vi "Cyclic Scheduler.vi"(8 "error in (no error)":errorcluster, 9 "timeout ms":i32=100, 11 "Variables":T1={"Process Ref"=refnum, "Comm Ref"=refnum, "Data Refs"={"ProtectionsAndCounters.Ref"=refnum, "Signals.Ref"=refnum, "Status.Ref"=refnum, "Overrides"=refnum, "IncomingSignals.Ref"=refnum, "CtrandProtctnVld.Ref"=refnum, "RcvTime.Ref"=refnum, "TimeDiff.Ref"=refnum, "IncomingProtCtr.Ref"=refnum}, "Settings"={"Name"="", "Priority"=0, "XNET Settings"={"Database"="", "Cluster"="", "Port"="", "Baud rate [Bd]"=0, "Termination"=0, "CAN I/O Mode"=0, "FD Baud rate [Bd]"=500000, "Priority"=100, "Use Legacy"=FALSE, "FD ISO Mode"=0, "Default Max Counter Value"=0.0, "Default Protect Type"=enum."Arb ID + Bytes Checksum with Inversion", "Include All Channels"=FALSE, "Scheduler Bucket Size"=10, "Scheduler Offset"=3}, "FPGA Session"=0, "Outgoing CAN Session"="", "Outgoing Cyclic Frame Count"=0, "Outgoing Cyclic Frames"=[], "Outgoing Event Frame Count"=0, "Outgoing Event Frames"=[], "Incoming CAN Session"="", "Incoming Frame Count"=0, "Incoming Frames"=[], "Incoming Values"={"Signal Values"=[], "Signal Invalid Values"=[], "ProtCtr Sig Values"=[], "Timestamps"=[], "Time Differences"=[], "IDs"=[]}}, "Stream Refs"={"Addon"="", "Port"="", "Filter Ref"=refnum, "Default Filter"={"ID Filters"=[], "Direction Filter"=enum."Tx/Rx", "Type Filter"=enum."All"}, "Port Settings"={"Mode"=0, "Baud Rate"=0, "Termination"=0, "FD ISO Mode"=0, "FD Baud Rate"=0}}, "Cyclic Scheduler Queue"=refnum, "Cyclic Scheduler FIFO"=refnum} {"Stream Refs"."Port Settings"."FD ISO Mode" items=["ISO", "Non ISO", "ISO Legacy"]; "Stream Refs"."Port Settings"."Termination" items=["Off", "On"]; "Stream Refs"."Port Settings"."Mode" items=["CAN 2.0", "CAN FD", "CAN FD+BRS"]; "Settings"."XNET Settings"."FD ISO Mode" items=["ISO", "Non ISO", "ISO Legacy"]; "Settings"."XNET Settings"."CAN I/O Mode" items=["CAN 2.0", "CAN FD", "CAN FD+BRS"]; "Settings"."XNET Settings"."Termination" items=["Off", "On"]}) -> (0 "error out":errorcluster)   [LabVIEW 2023, in "Protection and Counter Addon Engine.lvlib"]
uses:
  Protection and Counter Addon Engine.lvlib
  <vilib>/NI/NIVS Inline Async API/_VS Inline Async API/Process/Process.lvclass
  <vilib>/NI/NI VeriStand Addon Network Comm/Engine/VeriStand Comm.lvclass
  <vilib>/NI/NIVS Inline Async API/_Data Access Engine/Access Type Classes/Write/Write.lvclass
  <vilib>/NI/NIVS Inline Async API/_Data Access Engine/Access Type Classes/Read/Read.lvclass
  <vilib>/Platform/TimedLoop/XDataNode/XDataNode.xnode
  <vilib>/Platform/TimedLoop/XDataNode/nitl_modes.ctl
  <vilib>/Platform/TimedLoop/XDataNode/XDNodeRunTimeDep.lvlib
  <vilib>/Platform/TimedLoop/XDataNode/wakeup.ctl
  <vilib>/Platform/TimedLoop/XDataNode/timing_clust.ctl
  SubModules/Frame-Protection-Support/Source/Shared/Types/XNET Signal Configuration.ctl
  SubModules/Frame-Protection-Support/Source/Shared/Protection and Counter Support Shared.lvlib
  SubModules/Frame-Protection-Support/Source/Shared/Types/Protection Type.ctl
  Types/RT Async Engine Settings.ctl
  SubModules/Frame-Protection-Support/Source/Engine/Types/RT Protection Configuration.ctl
  SubModules/Frame-Protection-Support/Source/Engine/Protection and Counter Support Engine.lvlib
  SubModules/Frame-Protection-Support/Source/Engine/Types/RT Frame Settings.ctl
  <vilib>/NI/NIVS Inline Async API/_Data Access Engine/Data Access Engine/Types/Read.DVR.ctl
  <vilib>/NI/NIVS Inline Async API/_Data Access Engine/Data Access Engine/Data Access Engine.lvclass
  <vilib>/NI/NIVS Inline Async API/_Data Access Engine/Data Access Engine/Types/Write.DVR.ctl
  Types/RT Data References.ctl
  SubModules/Frame-Protection-Support/Source/Shared/Types/Exported Frame Type.ctl
  SubModules/Frame-Protection-Support/Source/Shared/Types/Exported Counter Settings.ctl
  SubModules/Frame-Protection-Support/Source/Shared/Types/Exported Event Trigger Type.ctl
  Types/RT Async Engine Variables.ctl
  SubModules/CAN-Streaming-Support/Source/Addon/Addon Shared/Types/Type Filter.ctl
  SubModules/CAN-Streaming-Support/Source/Addon/Addon Shared/CAN Stream Support Shared.lvlib
  SubModules/CAN-Streaming-Support/Source/Addon/Addon Shared/Types/Direction Filter.ctl
  SubModules/CAN-Streaming-Support/Source/Addon/Addon Shared/Types/Filter Parameters.ctl
  SubModules/CAN-Streaming-Support/Source/Addon/Addon Engine/Types/Engine Stream Refs.ctl
  SubModules/CAN-Streaming-Support/Source/Addon/Addon Engine/CAN Stream Support Engine.lvlib
  SubModules/CAN-Streaming-Support/Source/Addon/Addon Engine/Types/Engine Stream Port Settings.ctl
  Addon Shared/Types/XNET Settings.ctl
  Addon Shared/Protection and Counter Addon Shared.lvlib
  SubModules/Frame-Protection-Support/Source/Engine/Types/RT Frame Incoming Values.ctl
panel:
  out "Iteration Duration (ms)":i64
  out "Gen Period":u32
  out "Indices Enqueued":i32[](array[numeric])
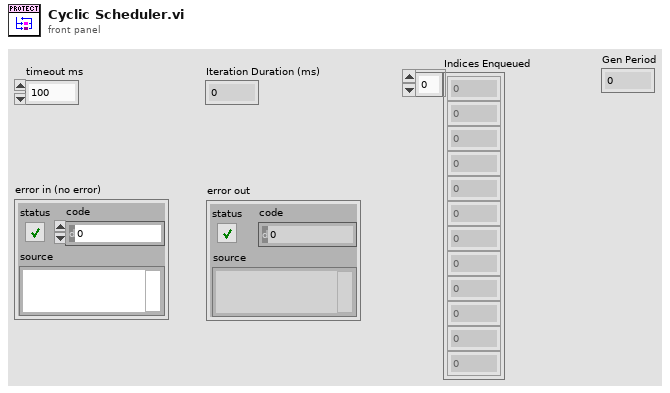
[diagram p1: front panel]
types:
  T1 = typedef "Protection and Counter Addon Engine.lvlib/RT Async Engine Variables.ctl" = cluster{"Process Ref":refnum<class "Process.lvclass">, "Comm Ref":refnum<class "VeriStand Comm.lvclass">, "Data Refs":T2, "Settings":T5, "Stream Refs":T15, "Cyclic Scheduler Queue":refnum<queue>, "Cyclic Scheduler FIFO":refnum<k33>}
  T2 = typedef "Protection and Counter Addon Engine.lvlib/RT Data References.ctl" = cluster{"ProtectionsAndCounters.Ref":T3, "Signals.Ref":T4, "Status.Ref":T3, "Overrides":T4, "IncomingSignals.Ref":T3, "CtrandProtctnVld.Ref":T3, "RcvTime.Ref":T3, "TimeDiff.Ref":T3, "IncomingProtCtr.Ref":T3}
  T3 = typedef "Data Access Engine.lvlib/Data Access Engine.lvclass/Write.DVR.ctl" = refnum<data-value>
  T4 = typedef "Data Access Engine.lvlib/Data Access Engine.lvclass/Read.DVR.ctl" = refnum<data-value>
  T5 = typedef "Protection and Counter Addon Engine.lvlib/RT Async Engine Settings.ctl" = cluster{"Name":string, "Priority":i32, "XNET Settings":T6, "FPGA Session":u32, "Outgoing CAN Session":refnum<k21>, "Outgoing Cyclic Frame Count":i32, "Outgoing Cyclic Frames":T8[], "Outgoing Event Frame Count":i32, "Outgoing Event Frames":T8[], "Incoming CAN Session":refnum<k21>, "Incoming Frame Count":i32, "Incoming Frames":T8[], "Incoming Values":T14}
  T6 = typedef "Protection and Counter Addon Shared.lvlib/XNET Settings.ctl" = cluster{"Database":refnum<k21>, "Cluster":refnum<k21>, "Port":string, "Baud rate [Bd]":u64, "Termination":u32, "CAN I/O Mode":u32, "FD Baud rate [Bd]":u64, "Priority":i32, "Use Legacy":bool, "FD ISO Mode":u32, "Default Max Counter Value":dbl, "Default Protect Type":T7, "Include All Channels":bool, "Scheduler Bucket Size":i32, "Scheduler Offset":i32}
  T7 = typedef "Protection and Counter Support Shared.lvlib/Protection Type.ctl" = enum16{"Arb ID + Bytes Checksum with Inversion", "Arb ID + Bytes CRC with Inversion", "Reversed Raw Signal Checksum with Inversion", "Concatenated Two's Compliment"}
  T8 = typedef "Protection and Counter Support Engine.lvlib/RT Frame Settings.ctl" = cluster{"Type":T9, "Frame ID":u32, "Payload Length":u32, "VS Offset":i32, "VS Length":i32, "Frame Conversion":refnum<k21>, "Frame.Data":dbl[], "Generation Period":u32, "Time Since Last Generation":u32, "Generation Iterations":u32, "Generation Counter":u32, "Has Protection?":bool, "Protection Configurations":T10[], "Has Counter?":bool, "Counter Configurations":T12[], "Has Disable?":bool, "Disable VS Index":i32, "Transmit Trigger":T13, "Trigger VS Index":i32}
  T9 = typedef "Protection and Counter Support Shared.lvlib/Exported Frame Type.ctl" = enum16{"Periodic", "Event", "Periodic/Event"}
  T10 = typedef "Protection and Counter Support Engine.lvlib/RT Protection Configuration.ctl" = cluster{"Protection Frame Index":i32, "Protection Type":T7, "Data Indeces":i32[], "Data Array":dbl[], "Check Sum Conversion":refnum<k21>, "CRC Channels":T11[], "Protection VS Index":i32, "Counter Data Index":i32, "Override Index":i32, "Override Value Index":i32}
  T11 = typedef "Protection and Counter Support Shared.lvlib/XNET Signal Configuration.ctl" = cluster{"Start Bit":i32, "Name":string, "Number of bits":i32, "Scale":dbl, "Offset":dbl, "Data Type":u32, "Counter":bool}
  T12 = typedef "Protection and Counter Support Shared.lvlib/Exported Counter Settings.ctl" = cluster{"Frame Index":i32, "Max Count":dbl, "VS Index":i32, "Bit Length":i64, "Override Index":i32, "Override Value Index":i32}
  T13 = typedef "Protection and Counter Support Shared.lvlib/Exported Event Trigger Type.ctl" = enum16{"Channel value change", "Trigger channel (not zero)", "Channel value change or trigger channel (not zero)", "Trigger channel (any value change)", "Channel value change or trigger channel (any value change)"}
  T14 = typedef "Protection and Counter Support Engine.lvlib/RT Frame Incoming Values.ctl" = cluster{"Signal Values":dbl[], "Signal Invalid Values":dbl[], "ProtCtr Sig Values":dbl[], "Timestamps":timestamp[], "Time Differences":dbl[], "IDs":u32[]}
  T15 = typedef "CAN Stream Support Engine.lvlib/Engine Stream Refs.ctl" = cluster{"Addon":string, "Port":refnum<k21>, "Filter Ref":refnum<data-value>, "Default Filter":T16, "Port Settings":T19}
  T16 = typedef "CAN Stream Support Shared.lvlib/Filter Parameters.ctl" = cluster{"ID Filters":u32[], "Direction Filter":T17, "Type Filter":T18}
  T17 = typedef "CAN Stream Support Shared.lvlib/Direction Filter.ctl" = enum16{"Tx/Rx", "Rx", "Tx"}
  T18 = typedef "CAN Stream Support Shared.lvlib/Type Filter.ctl" = enum16{"All", "CAN Data", "CAN Remote", "CAN Bus Error", "CAN 2.0 Data", "CAN FD Data", "CAN FD+BRS Data", "J1939 Data", "Delay", "Log Trigger", "Start Trigger"}
  T19 = typedef "CAN Stream Support Engine.lvlib/Engine Stream Port Settings.ctl" = cluster{"Mode":u32, "Baud Rate":u64, "Termination":u32, "FD ISO Mode":u32, "FD Baud Rate":u64}
  T20 = typedef "Protection and Counter Addon Engine.lvlib/RT Bucket of Indices.ctl" = cluster{"Counter":u32, "Gen Period":u32, "RT Indices":i32[]}
  T21 = typedef "XDNodeRunTimeDep.lvlib/timing_clust.ctl" = cluster{"Expected End [f-1]":u64, "Actual End [f-1]":u64, "Finished Late? [f-1]":bool, "Expected End [i-1]":u64, "Actual End [i-1]":u64, "Finished Late? [i-1]":bool, "Expected Start [i]":u64, "Actual Start [i]":u64, "Expected Start [f]":u64, "Actual Start [f]":u64, "Source Name":string, "Structure Name":string, "Period":i64, "Deadline":i64, "Offset":i64, "Start":i64, "Priority":i32, "Timeout":i32, "Mode":T22, "Wakeup Reason":T23, "Error":errorcluster, "Source Type":string, "Secondary Source Type":string, "Global End Time":u64, "Global Start Time":u64, "Frame Duration":u64, "Iteration Duration":u64, "Assigned CPU":i32, "I/O Scan Engine Mode":u32}
  T22 = typedef "XDNodeRunTimeDep.lvlib/nitl_modes.ctl" = enum32{"No Change", "Process missed periods, maintain original phase", "Discard missed periods, maintain original phase", "Process missed periods, ignore original phase", "Discard missed periods, ignore original phase"}
  T23 = typedef "XDNodeRunTimeDep.lvlib/wakeup.ctl" = enum32{"Normal", "Aborted", "Asynchronous wakeup", "Timing source error", "Timed loop error", "Timeout"}
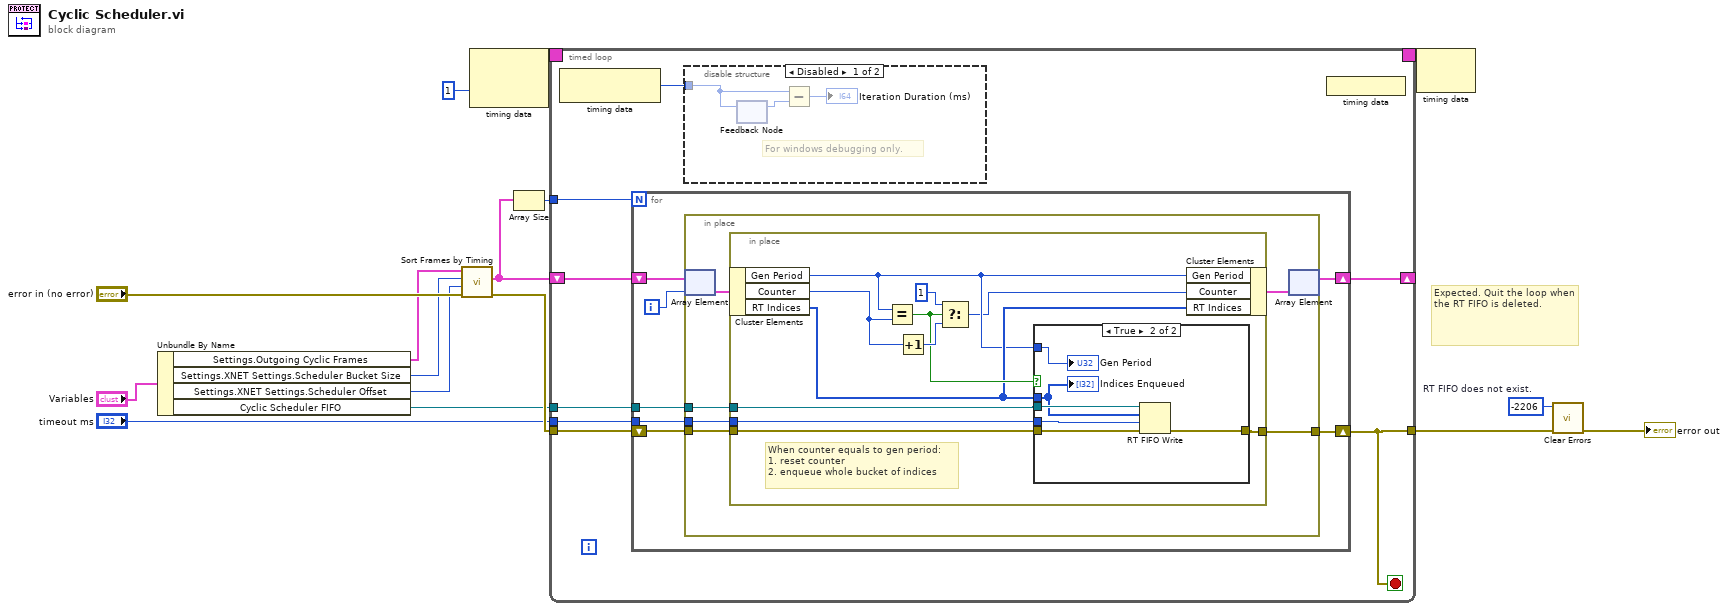
[diagram p0: block diagram]
diagram:
  w12 = -2206  # RT FIFO does not exist.
  # "Expected. Quit the loop when the RT FIFO is deleted."
  n1 = Unbundle By Name("Variables") -> ("Settings.Outgoing Cyclic Frames"=w1:T8[], "Settings.XNET Settings.Scheduler Bucket Size"=w2:i32, "Settings.XNET Settings.Scheduler Offset"=w3:i32, "Cyclic Scheduler FIFO"=w5:refnum<k33>)
  n2 = call "Sort Frames by Timing.vi"("error in (no error)"="error in (no error)", "Counter Offset"=w3, "Max frames per bucket"=w2, "Outgoing Cyclic Frames"=w1) -> ("error out"=w7:errorcluster, "Bucket of Indices"=w9:T20[])  [unwired: 5 in, 1 out]
  n3 = node-c288(i64 1 ("Period")) -> (w15:T21)  [unwired: 1 in]
  n4 = Array Size(array=w9) -> (size(s)=w8:i32)
  n5 = timed-loop {
    timing: w15 -> [_]
    timing-out: [_] -> w14
    shift-right: [w19] -> _
    shift-left: w9 -> [w24]
    tunnel: w8 -> [w23]
    tunnel: w5 -> [w22]
    tunnel: w7 -> [w21]
    tunnel: "timeout ms" -> [w20]
    tunnel: [w18] -> w4
    stop <- w18 stop-if-true
    n6 = node-c288() -> (w17:i64)  [unwired: 1 in]
    n7 = for {
      N: w23 -> [_]
      tunnel: w22 -> [w32]
      tunnel: w20 -> [w30]
      shift-right: [w28] -> w18
      shift-left: w21 -> [w31]
      shift-right: [w29] -> w19
      shift-left: w24 -> [w34]
      i -> [w33]
      n8 = in-place {
        in-place-border: w32 -> [w39]
        in-place-border: w31 -> [w38]
        in-place-border: w30 -> [w37]
        in-place-border: [w35] -> w28
        n9 = in-place-array #1(w34, w33) -> (w40:T20)
        n10 = in-place {
          in-place-border: w39 -> [w49]
          in-place-border: w38 -> [w48]
          in-place-border: w37 -> [w47]
          in-place-border: [w44] -> w35
          # "When counter equals to gen period:\n1. reset counter\n2. enqueue whole bucket of indices"
          n11 = in-place-cluster #2(w40) -> ("Gen Period"=w43:u32, "Counter"=w41:u32, "RT Indices"=w45:i32[])
          n12 = Equal?(x=w43, y=w41) -> (x = y?=w46:bool)
          n13 = Increment(x=w41) -> (x+1=w51:u32)
          n14 = Select(t=u32 1, s=w46, f=w51) -> (s? t:f=w42:u32)
          n15 = case shown="True" w46 {
            tunnel: w49 -> [_ w58]
            tunnel: w48 -> [w52 w57]
            tunnel: [w52 w56] -> w44
            tunnel: w47 -> [_ w55]
            tunnel: w45 -> [_ w54]
            tunnel: w43 -> [_ w53]
            frame False {
            }
            frame True {
              n16 = RT FIFO Write(0:w58, 1:w54, 2:w55, 3:w57) -> (11:w56:errorcluster)  [unwired: 1 in, 3 out]
              "Indices Enqueued" <- w54
              "Gen Period" <- w53
            }
          }
          n17 = in-place-cluster #2("Gen Period"=w43, "Counter"=w42, "RT Indices"=w45) -> (w36:T20)
        }
        n18 = in-place-array #1(w36) -> (w29:T20[])  [unwired: 1 out]
      }
    }
    n19 = disable-structure shown="Disabled" {
      disable-tunnel: w17 -> [w27 _]
      frame Disabled {
        # "For windows debugging only."
        n20 = feedback #3() -> (w26:i64)  [unwired: 1 in]
        n21 = feedback-in #3(w27) -> ()
        n22 = Subtract(x=w27, y=w26) -> (x-y=→"Iteration Duration (ms)":i64)
      }
      frame Enabled {
      }
    }
    n23 = node-c288() -> ()  [unwired: 1 out]
  }
  n24 = node-c288(w14) -> ()  [unwired: 1 out]
  n25 = call <vilib>:"Clear Errors.vi"("error in (no error)"=w4, "specific error code to clear (0: all)"=w12) -> ("error out"=→"error out":errorcluster)  [unwired: 4 in, 1 out]
